vi "update Keysight 9020A Correction Table Param.vi"(8 "error in (no error)":errorcluster, 10 "Keysight Correction Table":T1 {"Frequency (Hz)" format="%#_6p"}, 11 "Interface_Spectrum in":refnum<class "Interface_Spectrum.lvclass">) -> (0 "error out":errorcluster, 3 "Interface_Spectrum out":refnum<class "Interface_Spectrum.lvclass">)   [LabVIEW 2023, in "Spectrum Analyzer.lvlib" / "Interface_Spectrum.lvclass"]
uses:
  Interface_Spectrum.lvclass
  TYPE DEFINITION/Keysight 9020A/TYPE Keysight Correction Table Array.ctl
  Spectrum Analyzer.lvlib
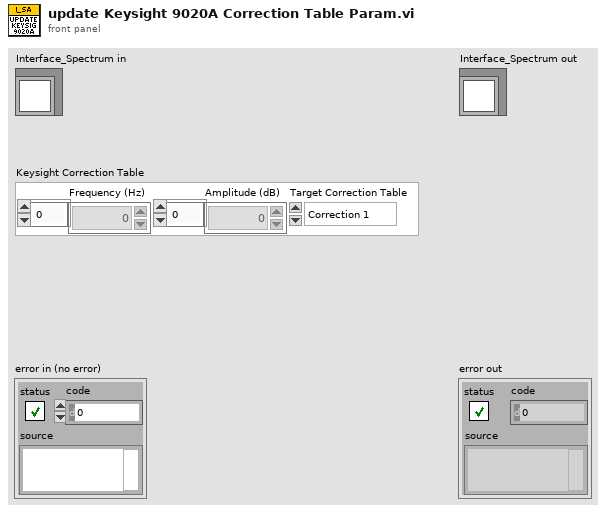
[diagram p1: front panel]
types:
  T1 = typedef "Spectrum Analyzer.lvlib/TYPE Keysight Correction Table Array.ctl" = cluster{"Frequency (Hz)":dbl[], "Amplitude (dB)":dbl[], "Target Correction Table":enum16{"Correction 1", "Correction 2", "Correction 3", "Correction 4", "Correction 5", "Correction 6", "Correction 7", "Correction 8"}}
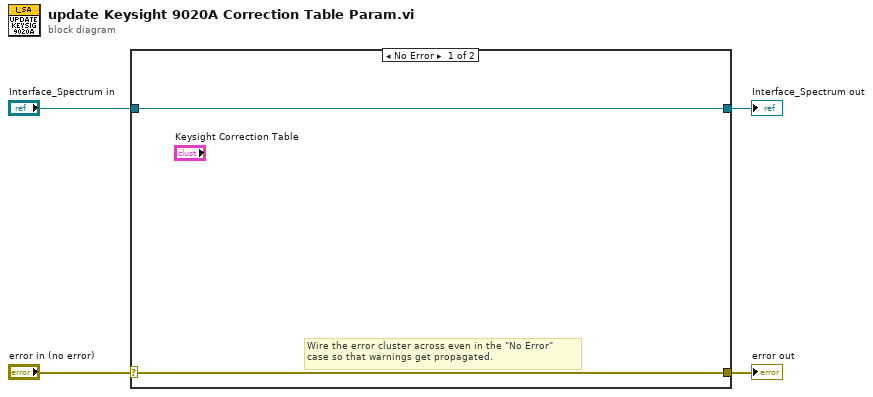
[diagram p0: block diagram]
diagram:
  n1 = case shown="No Error" "error in (no error)" {
    selector: "error in (no error)" -> [w5 w8]
    tunnel: [w5 w8] -> w3
    tunnel: [w6 w7] -> w1
    tunnel: "Interface_Spectrum in" -> [w6 w7]
    frame No Error {
      # "Wire the error cluster across even in the \"No Error\"\ncase so that warnings get propagated."
    }
    frame Error {
    }
  }
  "error out" <- w3
  "Interface_Spectrum out" <- w1
